vi "Temp_Formula (SubVI).vi"(2 "error in (no error)":errorcluster, 3 "In":dbl) -> (0 "error out":errorcluster, 1 "Out":dbl)   [LabVIEW 2024]
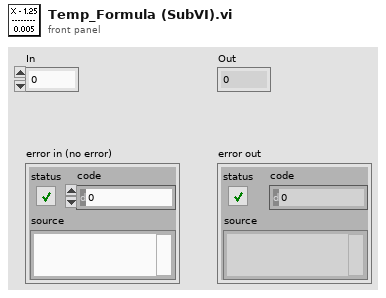
[diagram p1: front panel]
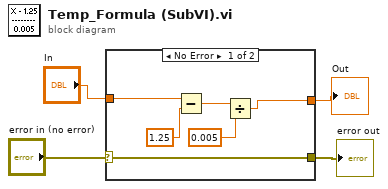
[diagram p0: block diagram]
diagram:
  n1 = case shown="No Error" "error in (no error)" {
    selector: "error in (no error)" -> [w7 w11]
    tunnel: [w7 w11] -> w2
    tunnel: "In" -> [w6 _]
    tunnel: [w5 _] -> w4
    frame No Error {
      n2 = Subtract(x=w6, y=1.25) -> (x-y=w9:dbl)
      n3 = Divide(x=w9, y=0.005) -> (x/y=w5:dbl)
    }
    frame Error {
    }
  }
  "error out" <- w2
  "Out" <- w4
